vi "SubscribeHeaterStateUpdated Send Stream.vi"(10 "Heater State":T1, 11 "Stream Data nin":T2={"gRPCid"=0, "Active"=FALSE, "timeout"=-1}) -> (0 "error out":errorcluster)   [LabVIEW 2020]
doc: "Send data with <b>Streaming?</b> parameter set to True to maintain stream active."
uses:
  Stream Data--cluster.ctl
  <vilib>/gRPC/LabVIEW gRPC Library/Shared/grpcId.ctl
  Program Files (x86)/National Instruments/LabVIEW 2020/examples/DQMH Consortium/DQMH Fundamentals - Thermal Chamber/Libraries/Thermal Chamber Controller_DQMH/Heater State--enum.ctl
  thermal-chamber-controller_server/RPC Messages/lv_python_grpc_webui_demo_v1_HeaterStateUpdated.ctl
  thermal-chamber-controller_server/RPC Messages/lv_python_grpc_webui_demo_v1_HeaterState.ctl
  thermal-chamber-controller_server/thermal-chamber-controller_server.lvlib
  thermal-chamber-controller_server/RPC Service/ThermalChamberController/ThermalChamberController.lvclass
  <vilib>/gRPC/LabVIEW gRPC Library/grpc-lvsupport-release.lvlib
  Program Files (x86)/National Instruments/LabVIEW 2020/examples/DQMH Consortium/DQMH Fundamentals - Thermal Chamber/Libraries/Thermal Chamber Controller_DQMH/Thermal Chamber Controller_DQMH.lvlib
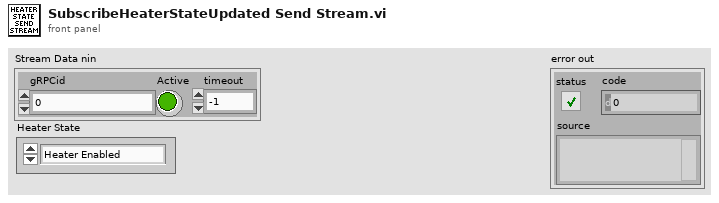
[diagram p1: front panel]
types:
  T1 = typedef "Thermal Chamber Controller_DQMH.lvlib/Heater State--enum.ctl" = enum16{"Heater Enabled", "Heater Disabled"}
  T2 = typedef "Stream Data--cluster.ctl" = cluster{"gRPCid":T3, "Active":bool, "timeout":i32}
  T3 = typedef "grpc-lvsupport-release.lvlib/grpcId.ctl" = u64
  T4 = typedef "thermal-chamber-controller_server.lvlib/lv_python_grpc_webui_demo_v1_HeaterStateUpdated.ctl" = cluster{"heater_state":T5}
  T5 = typedef "thermal-chamber-controller_server.lvlib/lv_python_grpc_webui_demo_v1_HeaterState.ctl" = enum32{"HEATER_ENABLED", "HEATER_DISABLED"}
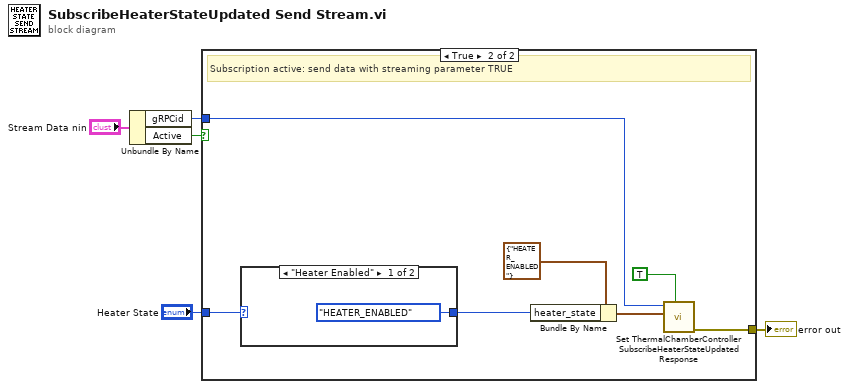
[diagram p0: block diagram]
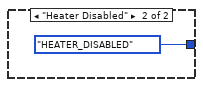
[diagram p3: hidden frame]
diagram:
  n1 = Unbundle By Name("Stream Data nin") -> ("gRPCid"=w5:T3, "Active"=w4:bool)
  n2 = case shown="True" w4 {
    tunnel: w5 -> [_ w11]
    tunnel: [_ w10] -> w1
    tunnel: "Heater State" -> [_ w7]
    frame False {
      # "Inactive: no action."
    }
    frame True {
      # "Subscription active: send data with streaming parameter TRUE"
      n3 = case shown="\"Heater Enabled\"" w7 {
        tunnel: [lv_python_grpc_webui_demo_v1_HeaterState."HEATER_ENABLED" ("heater_state") lv_python_grpc_webui_demo_v1_HeaterState."HEATER_DISABLED" ("heater_state")] -> w6
        frame "Heater Enabled" {
        }
        frame "Heater Disabled" {
        }
      }
      n4 = Bundle By Name(cluster=T4 {"heater_state"=enum."HEATER_ENABLED"} ("Message Data"), "heater_state"=w6) -> (w8:T4)
      n5 = call "Set ThermalChamberController SubscribeHeaterStateUpdated Response.vi"("Streaming? (F)"=TRUE, "Message Data"=w8, "gRPCid in"=w11) -> ("error out"=w10:errorcluster)  [unwired: 8 in]
    }
  }
  "error out" <- w1
